vi "UpdateElement(Single).vi"(7 "Qualified Name":string, 8 "error in (no error)":errorcluster, 9 "Value":string, 10 "Key":string, 11 "ConfigManager.Text in":refnum<class "ConfigManager.Text.lvclass">) -> (0 "error out":errorcluster, 3 "ConfigManager.Text out":refnum<class "ConfigManager.Text.lvclass">)   [LabVIEW 2013, in "CfgManager.Text.lvlib" / "ConfigManager.Text.lvclass"]
uses:
  ConfigManager.Text.lvclass
  Update -- cluster.ctl
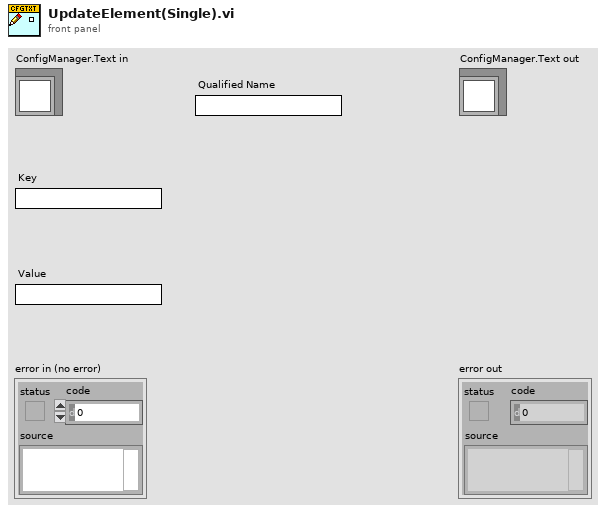
[diagram p1: front panel]
types:
  T1 = typedef "CfgManager.Text.lvlib/ConfigManager.Text.lvclass/Update -- cluster.ctl" = cluster{"Qualified Name":string[], "Keys":string[], "Values":string[]}
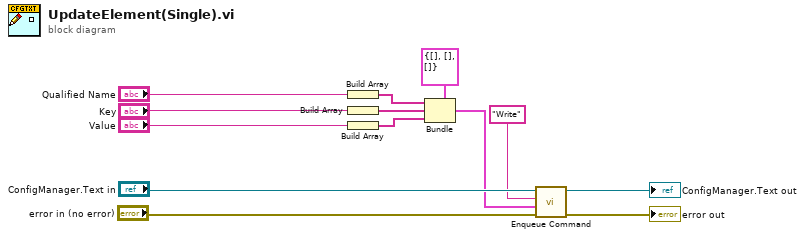
[diagram p0: block diagram]
diagram:
  n1 = Build Array("Qualified Name") -> (w1:string[])
  n2 = Build Array("Key") -> (w6:string[])
  n3 = Build Array("Value") -> (w2:string[])
  n4 = Bundle(cluster=T1 {"Qualified Name"=[], "Keys"=[], "Values"=[]} ("Update"), "Qualified Name"=w1, "Keys"=w6, "Values"=w2) -> (w4:T1)
  n5 = call "Enqueue Command.vi"("error in (no error)"="error in (no error)", "args"=w4, "command"="Write", "ConfigManager.Text in"="ConfigManager.Text in") -> ("error out"=→"error out":errorcluster, "ConfigManager.Text out"=→"ConfigManager.Text out":refnum<class "ConfigManager.Text.lvclass">)  [unwired: 5 in, 1 out]
